vi "Synthf2700.vi"(11 "Frequency in MHz":string="f2712.54") -> ()   [LabVIEW 2024]
uses:
  Serial Port.vi
  <vilib>/Instr/_visa.llb/VISA Configure Serial Port (Instr).vi
panel:
  out "read buffer":string
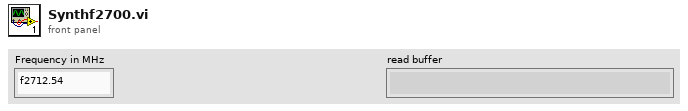
[diagram p1: front panel]
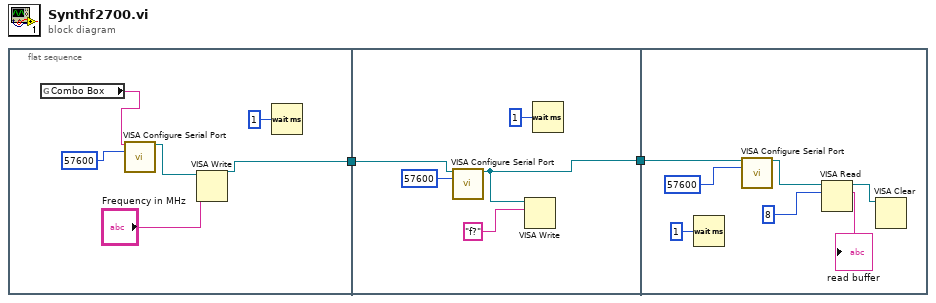
[diagram p0: block diagram]
diagram:
  n1 = flat-sequence {
    tunnel: [w4] -> w1
    tunnel: [w10] -> w2
    tunnel: w1 -> [w9]
    tunnel: w2 -> [w14]
    frame #0 {
      n2 = global read "Serial Port.vi" "Combo Box"() -> (w3:string)
      n3 = call-poly "VISA Configure Serial Port"("VISA resource name"=w3, "baud rate (9600)"=u32 57600) -> ("VISA resource name out"=w7:refnum<visa-resource-name>)  [unwired: 12 in, 1 out]
      n4 = VISA Write(VISA resource name=w7, write buffer="Frequency in MHz") -> (VISA resource name out=w4:refnum<visa-resource-name>)  [unwired: 1 in, 2 out]
      n5 = Wait (ms)(milliseconds to wait=u32 1) -> ()  [unwired: 1 out]
    }
    frame #1 {
      n6 = call-poly "VISA Configure Serial Port"("VISA resource name"=w9, "baud rate (9600)"=u32 57600) -> ("VISA resource name out"=w10:refnum<visa-resource-name>)  [unwired: 12 in, 1 out]
      n7 = VISA Write(VISA resource name=w10, write buffer="f?") -> ()  [unwired: 1 in, 3 out]
      n8 = Wait (ms)(milliseconds to wait=u32 1) -> ()  [unwired: 1 out]
    }
    frame #2 {
      n9 = Wait (ms)(milliseconds to wait=u32 1) -> ()  [unwired: 1 out]
      n10 = call-poly "VISA Configure Serial Port"("VISA resource name"=w14, "baud rate (9600)"=u32 57600) -> ("VISA resource name out"=w19:refnum<visa-resource-name>)  [unwired: 12 in, 1 out]
      n11 = VISA Read(VISA resource name=w19, byte count=u32 8) -> (VISA resource name out=w16:refnum<visa-resource-name>, read buffer=→"read buffer":string)  [unwired: 1 in, 2 out]
      n12 = VISA Clear(VISA resource name=w16) -> ()  [unwired: 1 in, 2 out]
    }
  }
